vi "VI Tree.vi"   [LabVIEW 2026, in "RSysUtils Array.lvlib"]
doc: "VI Tree\nThis VI lists all the public VIs and CTLs of the library."
uses:
  RSysUtils Array.lvlib
  ba1bf76e-467c-49ce-86b9-cc5a3a6e2ce2.vi
  458117f3-955c-4287-a7ef-38def727e367.vi
  f31cf8c2-0961-47cd-bb5c-73e886d5015f.vi
  7b3340ea-90ca-4731-b4eb-5a0cf926790f.vi
  38754230-f1a7-4146-a332-b9cd7aba1977.vi
  09724e98-836f-4526-b2fb-3e63d74d26a7.vi
  17322ae4-9ef5-48dd-82ae-52511072bfb0.vi
  94493d89-0741-439a-b558-772d7de2f4d8.vi
  7bccd967-131f-4dc5-a5bc-aaefe1a1eff7.vi
  cabd316d-0c25-456e-850d-cd565cbe56fa.vi
  d2b69910-5420-468b-9776-ad4572d0d405.vi
  dd02bd8f-cd92-498b-90e8-a9babf38ad6e.vi
  4545d936-58fc-4f8a-9ac4-6f1cbb87b806.vi
  867cb03c-256a-44eb-aeb4-c247efdc2744.vi
  485f5e7c-b6a7-4a81-901a-e2efb5c5f5c7.vi
  c034a3f1-509f-4893-bf9d-c77e19edf2b8.vi
  c15041a7-6b69-4ceb-bc85-0e522fb3b349.vi
  631338d5-e1e1-4f52-ae29-67feeded1cd7.vi
  71443069-4016-4995-b90c-136c16faba5c.vi
  f312710d-7260-4e19-934b-9d4e5d848ab1.vi
  2d6446b1-0283-4cbf-917a-1b84e0d281ef.vi
  b667c1fa-328b-413f-b78e-017b45a49bc9.vi
  402da9ed-e4a3-49d0-8d83-356117078460.vi
  812f68fc-c84f-4db0-80b1-00b8706695cd.vi
  3f01d68a-5210-42de-a0ed-5209d1ee7da6.vi
panel:
  # "VI Tree\nSee the block diagram for the VI Tree"
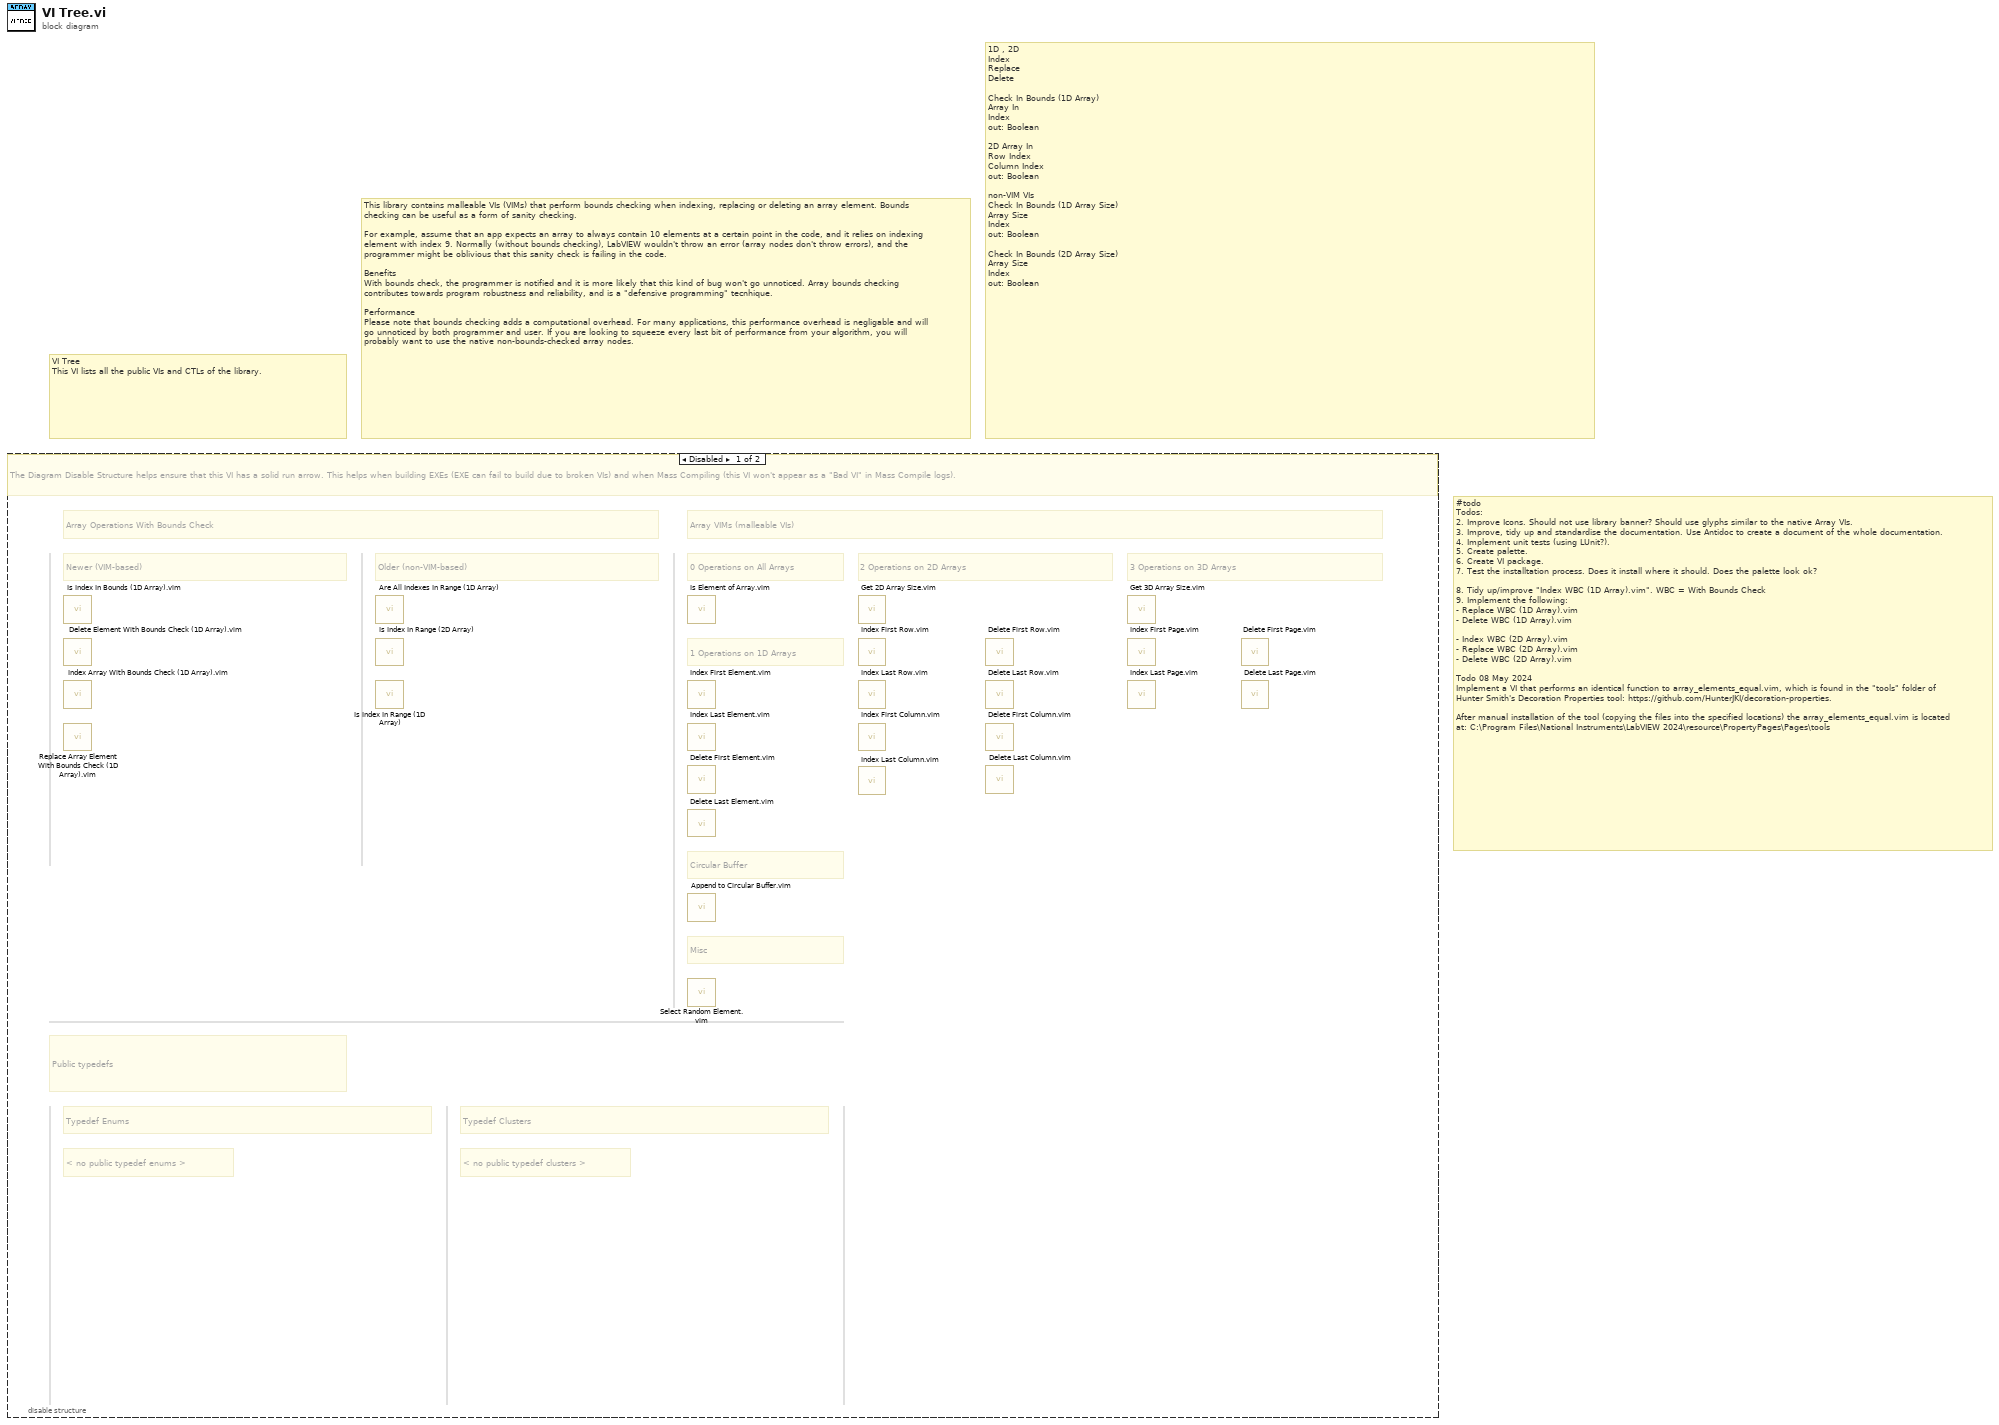
[diagram p0: block diagram]
diagram:
  # "#todo\nTodos:\n2. Improve Icons. Should not use library banner? Should use glyphs similar to the native Array VIs.\n3. Improve, tidy up and standardise the documentation. Use Antidoc to create a document of the whole documentation.\n4. Implement unit tests (using LUnit?).\n5. Create palette.\n6. Create VI package.\n7. Test the installtation process. Does it install where it should. Does the palette look ok?\n\n8. Tidy up/improve \"Index WBC (1D Array).vim\". WBC = With Bounds Check\n9. Implement the following:\n- Replace WBC (1D Array).vim\n- Delete WBC (1D Array).vim\n\n- Index WBC (2D Array).vim\n- Replace WBC (2D Array).vim\n- Delete WBC (2D Array).vim\n\nTodo 08 May 2024\nImplement a VI that performs an identical function to array_elements_equal.vim, which is found in the \"tools\" folder of Hunter Smith's Decoration Properties tool: https://github.com/HunterJKI/decoration-properties.\n\nAfter manual installation of the tool (copying the files into the specified locations) the array_elements_equal.vim is located at: C:\\Program Files\\National Instruments\\LabVIEW 2024\\resource\\PropertyPages\\Pages\\tools"
  # "1D , 2D\nIndex\nReplace\nDelete\n\nCheck In Bounds (1D Array)\nArray In\nIndex\nout: Boolean\n\n2D Array In\nRow Index\nColumn Index\nout: Boolean\n\nnon-VIM VIs\nCheck In Bounds (1D Array Size)\nArray Size\nIndex\nout: Boolean\n\nCheck In Bounds (2D Array Size)\nArray Size\nIndex\nout: Boolean"
  # "This library contains malleable VIs (VIMs) that perform bounds checking when indexing, replacing or deleting an array element. Bounds checking can be useful as a form of sanity checking. \n\nFor example, assume that an app expects an array to always contain 10 elements at a certain point in the code, and it relies on indexing element with index 9. Normally (without bounds checking), LabVIEW wouldn't throw an error (array nodes don't throw errors), and the programmer might be oblivious that this sanity check is failing in the code.\n\nBenefits\nWith bounds check, the programmer is notified and it is more likely that this kind of bug won't go unnoticed. Array bounds checking contributes towards program robustness and reliability, and is a \"defensive programming\" tecnhique.\n\nPerformance\nPlease note that bounds checking adds a computational overhead. For many applications, this performance overhead is negligable and will go unnoticed by both programmer and user. If you are looking to squeeze every last bit of performance from your algorithm, you will probably want to use the native non-bounds-checked array nodes."
  # "VI Tree\nThis VI lists all the public VIs and CTLs of the library."
  n1 = disable-structure shown="Disabled" {
    frame Disabled {
      # "Misc"
      # "3 Operations on 3D Arrays"
      # "Circular Buffer"
      # "2 Operations on 2D Arrays"
      # "1 Operations on 1D Arrays"
      # "Array VIMs (malleable VIs)"
      # "Array Operations With Bounds Check"
      # "0 Operations on All Arrays"
      # "Older (non-VIM-based)"
      # "Newer (VIM-based)"
      # "< no public typedef enums >"
      # "< no public typedef clusters >"
      # "Typedef Clusters"
      # "Typedef Enums"
      # "Public typedefs"
      # "The Diagram Disable Structure helps ensure that this VI has a solid run arrow. This helps when building EXEs (EXE can fail to build due to broken VIs) and when Mass Compiling (this VI won't appear as a \"Bad VI\" in Mass Compile logs)."
      n2 = call "Is Index In Bounds (1D Array).vim"() -> ()  [unwired: 2 in, 1 out]
      n3 = call "Delete Element With Bounds Check (1D Array).vim"() -> ()  [unwired: 10 in, 2 out]
      n4 = call "Index Array With Bounds Check (1D Array).vim"() -> ()  [unwired: 10 in, 2 out]
      n5 = call "Replace Array Element With Bounds Check (1D Array).vim"() -> ()  [unwired: 10 in, 2 out]
      n6 = call "Are All Indexes In Range (1D Array).vi"() -> ()  [unwired: 2 in, 1 out]
      n7 = call "Is Index In Range (2D Array).vi"() -> ()  [unwired: 3 in, 1 out]
      n8 = call "Is Index In Range (1D Array).vi"() -> ()  [unwired: 2 in, 1 out]
      n9 = call "Is Element of Array.vim"() -> ()  [unwired: 2 in, 1 out]
      n10 = call "Index First Element.vim"() -> ()  [unwired: 1 in, 1 out]
      n11 = call "Index Last Element.vim"() -> ()  [unwired: 1 in, 1 out]
      n12 = call "Delete First Element.vim"() -> ()  [unwired: 2 in, 2 out]
      n13 = call "Delete Last Element.vim"() -> ()  [unwired: 2 in, 2 out]
      n14 = call "Append to Circular Buffer.vim"() -> ()  [unwired: 3 in, 3 out]
      n15 = call "Select Random Element.vim"() -> ()  [unwired: 1 in, 1 out]
      n16 = call "Get 2D Array Size.vim"() -> ()  [unwired: 1 in, 2 out]
      n17 = call "Index First Row.vim"() -> ()  [unwired: 1 in, 1 out]
      n18 = call "Index Last Row.vim"() -> ()  [unwired: 1 in, 1 out]
      n19 = call "Index First Column.vim"() -> ()  [unwired: 1 in, 1 out]
      n20 = call "Index Last Column.vim"() -> ()  [unwired: 1 in, 1 out]
      n21 = call "Delete First Row.vim"() -> ()  [unwired: 2 in, 2 out]
      n22 = call "Delete Last Row.vim"() -> ()  [unwired: 2 in, 2 out]
      n23 = call "Delete First Column.vim"() -> ()  [unwired: 2 in, 2 out]
      n24 = call "Delete Last Column.vim"() -> ()  [unwired: 2 in, 2 out]
      n25 = call "Get 3D Array Size.vim"() -> ()  [unwired: 1 in, 3 out]
      n26 = call "Index First Page.vim"() -> ()  [unwired: 1 in, 1 out]
      n27 = call "Index Last Page.vim"() -> ()  [unwired: 1 in, 1 out]
      n28 = call "Delete First Page.vim"() -> ()  [unwired: 2 in, 2 out]
      n29 = call "Delete Last Page.vim"() -> ()  [unwired: 2 in, 2 out]
    }
    frame Enabled {
    }
  }
